vi "Try It.vi"(8 "error in":errorcluster, 10 "Main Demo UI":refnum<vi>, 11 "Demo":refnum<class "Demo.lvclass">) -> (0 "error out":errorcluster)   [LabVIEW 2020]
uses:
  Demo_class/Demo.lvclass
  Demo_class/Demo.lvclass/Demo.ctl
  <vilib>/Utility/traverseref.llb/VI Scripting - Traverse.lvlib
  <vilib>/Utility/traverseref.llb/TRef TravTarget.ctl
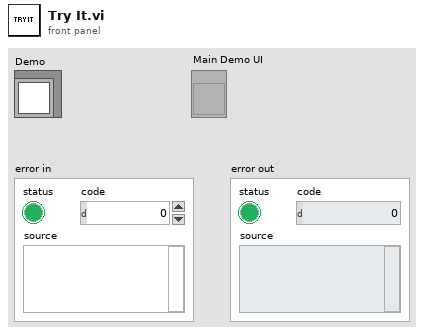
[diagram p1: front panel]
types:
  T1 = typedef "TRef TravTarget.ctl" = enum16{"FP", "BD", "Other"}
  T2 = enum32{"Invalid", "Standard", "Closed", "Hidden", "Minimized", "Maximized"}
  T3 = typedef "LVRectTypeDef.ctl" = cluster{"Left":i16, "Top":i16, "Right":i16, "Bottom":i16}
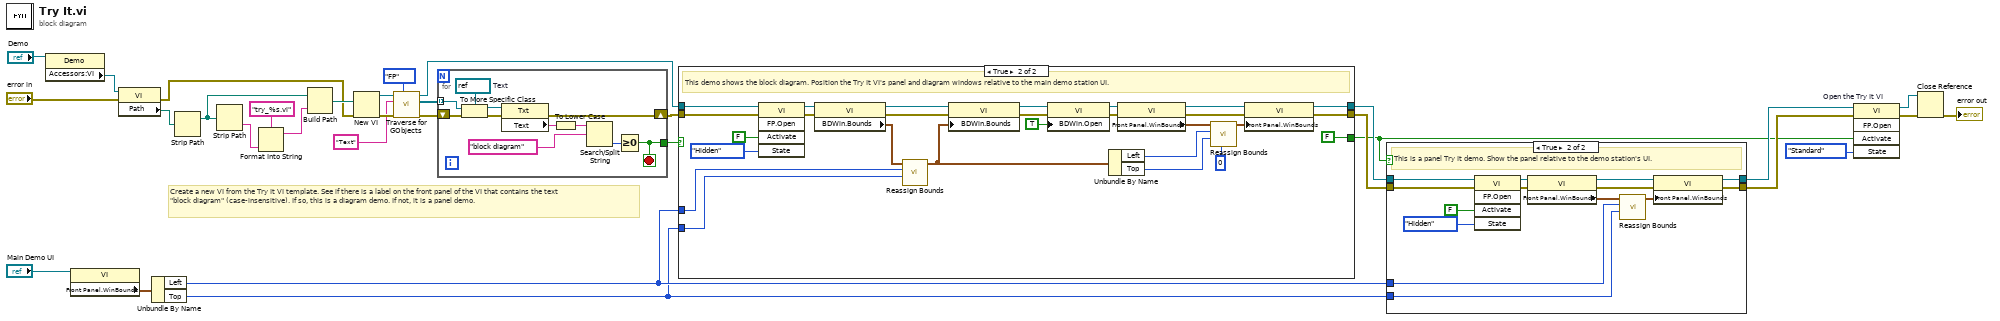
[diagram p0: block diagram]
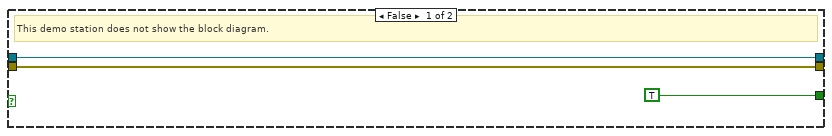
[diagram p2: hidden frame]
diagram:
  # "Create a new VI from the Try It VI template. See if there is a label on the front panel of the VI that contains the text \"block diagram\" (case-insensitive). If so, this is a diagram demo. If not, it is a panel demo."
  n1 = property class="Demo"(reference="Demo") -> ("Accessors:VI"=w30:refnum<vi>)  [unwired: 1 in, 2 out]
  n2 = property class="VI"(reference="Main Demo UI") -> ("Front Panel.WinBounds"=w8:T3)  [unwired: 1 in, 2 out]
  n3 = property class="VI"(reference=w30, error in="error in") -> (error out=w23:errorcluster, "Path"=w29:path)  [unwired: 1 out]
  n4 = Unbundle By Name(w8) -> ("Left"=w2:i16, "Top"=w1:i16)
  n5 = Strip Path(path=w29) -> (stripped path=w28:path)  [unwired: 1 out]
  n6 = Strip Path(path=w28) -> (name=w26:string)  [unwired: 1 out]
  n7 = Format Into String(format string="try_%s.vi", w26) -> (resulting string=w25:string)  [unwired: 2 in, 1 out]
  n8 = Build Path(base path=w28, name or relative path=w25) -> (appended path=w24:path)
  n9 = New VI(8:w23, 10:w24) -> (0:w22:errorcluster, 3:w17:refnum<vi>)  [unwired: 5 in]
  n10 = call <vilib>:"Traverse for GObjects.vi"("Traverse Target"=TRef_TravTarget."FP", "error in (no error)"=w22, "Class Name"="Text", "VI Refnum"=w17) -> ("error out"=w14:errorcluster, "References"=w13:refnum<vi>[], "dup VI Refnum"=w10:refnum<vi>)  [unwired: 4 in, 1 out]
  n11 = for {
    shift-right: [w33] -> w11
    shift-left: w14 -> [w43]
    tunnel: w13 -> [w42] mode=indexing
    tunnel: [w34] -> w12
    stop <- w34 stop-if-true
    w41 = refnum<vi> refnum  # Text
    n12 = To More Specific Class(target class=w41, reference=w42, error in=w43) -> (specific class reference=w39:refnum<vi>, error out=w40:errorcluster)
    n13 = property class="Txt"(reference=w39, error in=w40) -> (error out=w33:errorcluster, "Text"=w38:string)  [unwired: 1 out]
    n14 = To Lower Case(string=w38) -> (all lower case string=w36:string)
    n15 = Search/Split String(string=w36, search string/char (-)="block diagram") -> (offset of match=w35:i32)  [unwired: 1 in, 2 out]
    n16 = Greater Or Equal To 0?(x=w35) -> (x >= 0?=w34:bool)
  }
  n17 = case shown="True" w12 {
    tunnel: [w45 w69] -> w7
    tunnel: [w46 w67] -> w5
    tunnel: w11 -> [w45 w66]
    tunnel: w10 -> [w46 w65]
    tunnel: [TRUE ("Activate?") FALSE ("Activate?")] -> w3
    tunnel: w2 -> [_ w53]
    tunnel: w1 -> [_ w52]
    frame False {
      # "This demo station does not show the block diagram."
    }
    frame True {
      # "This demo shows the block diagram. Position the Try It VI's panel and diagram windows relative to the main demo station UI."
      n18 = invoke class="VI" method="FP.Open"(reference=w65, error in=w66, "Activate"=FALSE ("Activate?"), "State"=T2."Hidden") -> (reference out=w60:refnum<vi>, error out=w59:errorcluster)  [unwired: 1 in, 3 out]
      n19 = property class="VI"(reference=w60, error in=w59) -> (reference out=w63:refnum<vi>, error out=w62:errorcluster, "BDWin.Bounds"=w61:T3)
      n20 = call "Reassign Bounds.vi"("New Top"=w52, "New Left"=w53, "Bounds in"=w61) -> ("Bounds out"=w54:T3)  [unwired: 8 in]
      n21 = property class="VI"(reference=w63, error in=w62, "BDWin.Bounds"=w54) -> (reference out=w57:refnum<vi>, error out=w58:errorcluster)
      n22 = property class="VI"(reference=w57, error in=w58, "BDWin.Open"=TRUE ("Block Diagram Window:Open")) -> (reference out=w55:refnum<vi>, error out=w56:errorcluster)
      n23 = Unbundle By Name(w54) -> ("Left"=w49:i16, "Top"=w48:i16)
      n24 = property class="VI"(reference=w55, error in=w56) -> (reference out=w68:refnum<vi>, error out=w70:errorcluster, "Front Panel.WinBounds"=w51:T3)
      n25 = call "Reassign Bounds.vi"("Offset from New (100)"=i16 0, "New Top"=w48, "New Left"=w49, "Bounds in"=w51) -> ("Bounds out"=w50:T3)  [unwired: 7 in]
      n26 = property class="VI"(reference=w68, error in=w70, "Front Panel.WinBounds"=w50) -> (reference out=w67:refnum<vi>, error out=w69:errorcluster)
    }
  }
  n27 = case shown="True" w3 {
    tunnel: w7 -> [w74 w83]
    tunnel: [w74 w82] -> w6
    tunnel: w5 -> [w75 w81]
    tunnel: [w75 w80] -> w4
    tunnel: w2 -> [_ w77]
    tunnel: w1 -> [_ w76]
    frame False {
      # "This is a diagram Try It demo. Its panel and diagram have already been shown."
    }
    frame True {
      # "This is a panel Try It demo. Show the panel relative to the demo station's UI."
      n28 = invoke class="VI" method="FP.Open"(reference=w81, error in=w83, "Activate"=FALSE ("Activate?"), "State"=T2."Hidden") -> (reference out=w87:refnum<vi>, error out=w86:errorcluster)  [unwired: 1 in, 3 out]
      n29 = property class="VI"(reference=w87, error in=w86) -> (reference out=w85:refnum<vi>, error out=w84:errorcluster, "Front Panel.WinBounds"=w79:T3)
      n30 = call "Reassign Bounds.vi"("New Top"=w76, "New Left"=w77, "Bounds in"=w79) -> ("Bounds out"=w78:T3)  [unwired: 8 in]
      n31 = property class="VI"(reference=w85, error in=w84, "Front Panel.WinBounds"=w78) -> (reference out=w80:refnum<vi>, error out=w82:errorcluster)
    }
  }
  n32 = invoke on="Open the Try It VI" class="VI" method="FP.Open"(reference=w4, error in=w6, "Activate"=w3, "State"=T2."Standard") -> (reference out=w19:refnum<vi>, error out=w20:errorcluster)  [unwired: 1 in, 3 out]
  n33 = Close Reference(reference=w19, error in (no error)=w20) -> (error out=→"error out":errorcluster)
